vi "Close.vi"(8 "error in (no error)":errorcluster, 11 "Tektronix MSO5 in":refnum<class "Tektronix MSO5.lvclass">) -> (0 "error out":errorcluster, 3 "Tektronix MSO5 out":refnum<class "Tektronix MSO5.lvclass">)   [LabVIEW 2025, in "Scope.lvlib" / "Tektronix MSO5.lvclass"]
uses:
  Tektronix MSO5.lvclass
  Tektronix MSO5.lvclass/Tektronix MSO5.ctl
  <instrlib>/Tektronix MSO5X Series/Tektronix MSO5X Series.lvlib
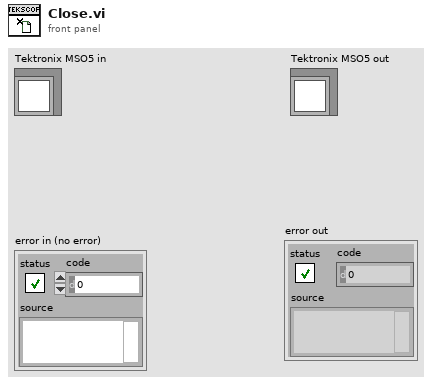
[diagram p1: front panel]
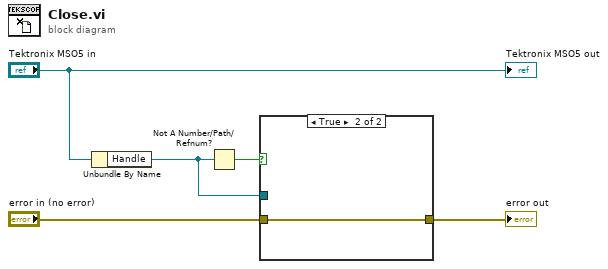
[diagram p0: block diagram]
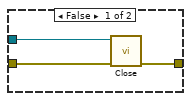
[diagram p2: hidden frame]
diagram:
  n1 = Unbundle By Name("Tektronix MSO5 in") -> ("Handle"=w2:refnum<visa-resource-name>)
  n2 = Not A Number/Path/Refnum?(number/path/refnum=w2) -> (NaN/Path/Refnum?=w1:bool)
  n3 = case shown="True" w1 {
    tunnel: [w6 w9] -> w5
    tunnel: "error in (no error)" -> [w7 w9]
    tunnel: w2 -> [w8 _]
    frame False {
      n4 = call <instrlib>:"Close.vi"("error in (no error)"=w7, "VISA resource name"=w8) -> ("error out"=w6:errorcluster)  [unwired: 9 in]
    }
    frame True {
    }
  }
  "error out" <- w5
  "Tektronix MSO5 out" <- "Tektronix MSO5 in"
